vi "Send Registration Event.vi"(4 "line limit":i32, 6 "log limit":i32, 8 "error in (no error)":errorcluster, 9 "auto-scroll":bool, 10 "ctl ref":refnum<vi>, 11 "handler name":string) -> (0 "error out":errorcluster)   [LabVIEW 2018, in "GLog.lvlib" / "UI Updater.lvlib"]
uses:
  UI Updater.lvlib
  Events/Register.ctl
  <vilib>/event_ctls.llb/usereventprio.ctl
panel:
  # "Connector Pane"
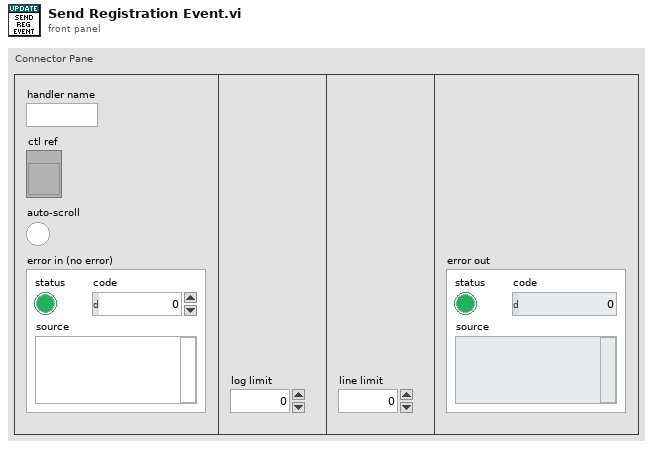
[diagram p1: front panel]
types:
  T1 = typedef "usereventprio.ctl" = enum32{"high priority", "normal priority"}
  T2 = typedef "GLog.lvlib/UI Updater.lvlib/Register.ctl" = cluster{"Handler Name":string, "Ctl Ref":refnum<vi>, "Log Limit":i32, "Line Limit":i32, "AutoScroll?":bool}
  T3 = typedef "GLog.lvlib/UI Updater.lvlib/Events.ctl" = cluster{"Write Log":refnum<user-event>, "Register":refnum<user-event>, "Unregister":refnum<user-event>}
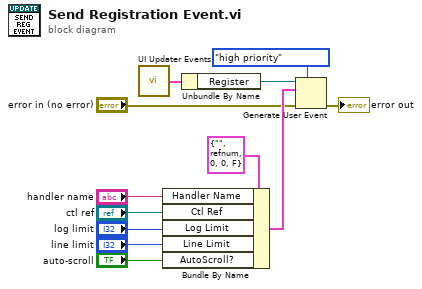
[diagram p0: block diagram]
diagram:
  n1 = call "UI Updater Events.vi"() -> ("UI Updater"=w3:T3)  [unwired: 1 in]
  n2 = Bundle By Name(cluster=T2 {"Handler Name"="", "Ctl Ref"=refnum, "Log Limit"=0, "Line Limit"=0, "AutoScroll?"=FALSE} ("event data"), "Handler Name"="handler name", "Ctl Ref"="ctl ref", "Log Limit"="log limit", "Line Limit"="line limit", "AutoScroll?"="auto-scroll") -> (w8:T2)
  n3 = Unbundle By Name(w3) -> ("Register"=w4:refnum<user-event>)
  n4 = Generate User Event(priority (normal)=usereventprio."high priority", user event=w4, event data cluster=w8, error in="error in (no error)") -> (error out=→"error out":errorcluster)  [unwired: 1 out]
